vi "VIH - CHM Project - Write TOC File - Add TOC Record - Get Palette Items.vi"(7 "Project Files":T3, 8 "error in":errorcluster, 11 "Palette Menu Path":path) -> (0 "error out":errorcluster, 2 "Items":T2(array[cluster]), 3 "dup Palette Menu Path":path)   [LabVIEW 2014]
doc: "::: VI Helpeks :::\nCopyright (c) 2000-2026 Konstantin Shifershteyn. All rights reserved."
uses:
  _VIH HelpGen - Palette.llb/VIH HelpGen Typedef - Palette - Item Type Enum.ctl
panel:
  # "VI Helpeks\nCopyright (c) 2012-2026 Konstantin Shifershteyn"
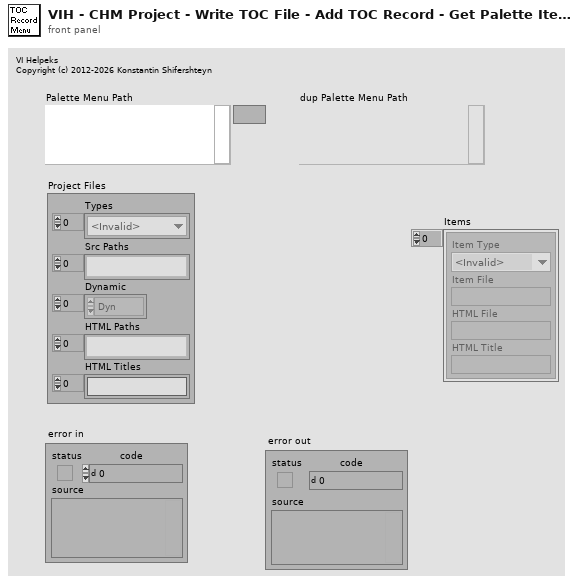
[diagram p1: front panel]
types:
  T1 = typedef "VIH HelpGen Typedef - Palette - Item Type Enum.ctl" = enum32{"<Invalid>", "<unknown>", "VI", "Menu", "LV Func", "Express VI", "Poly VI", "CTL", "HTML"}
  T2 = cluster{"Item Type":T1, "Item File":path, "HTML File":path, "HTML Title":string}[]
  T3 = cluster{"Types":T1[], "Src Paths":path[], "Dynamic":enum16{"Dyn", "Stat", "Both"}[], "HTML Paths":path[], "HTML Titles":string[]}
  T4 = typedef "VIH HelpGen Typedef - Palette - Item Info Cluster.ctl" = cluster{"Item Type":T1, "Item Name":string, "Item File":path, "Parent palette":path, "Not found":bool}
  T5 = cluster{"Item Type":T1, "Item File":path, path, string}
  T6 = cluster{"Item Type":T1, "Item File":path, "HTML File":path, "HTML Title":string}
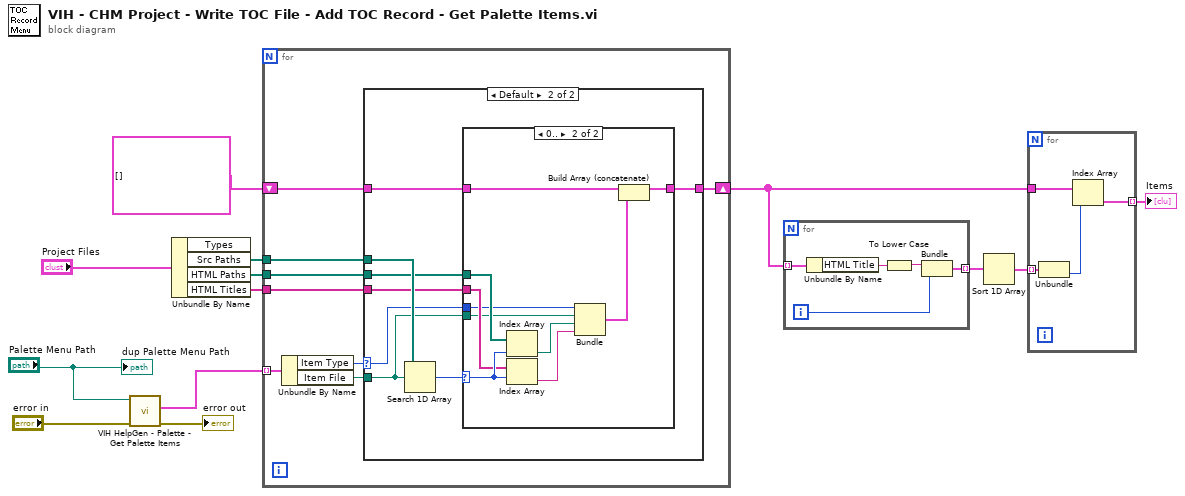
[diagram p0: block diagram]
diagram:
  n1 = call "VIH HelpGen - Palette - Get Palette Items.vi"("error in"="error in", "Palette Path"="Palette Menu Path") -> ("error out"=→"error out":errorcluster, "Items Array"=w10:T4[])  [unwired: 7 in, 1 out]
  n2 = Unbundle By Name("Project Files") -> ("Src Paths"=w9:path[], "HTML Paths"=w6:path[], "HTML Titles"=w7:string[])  [unwired: 1 out]
  n3 = for {
    tunnel: w10 -> [w21] mode=indexing
    tunnel: w9 -> [w18]
    tunnel: w7 -> [w17]
    tunnel: w6 -> [w16]
    shift-right: [w14] -> w3
    shift-left: T2 [] -> [w15]
    n4 = Unbundle By Name(w21) -> ("Item Type"=w20:T1, "Item File"=w19:path)
    n5 = case shown="Default" w20 {
      selector: w20 -> [_ w26]
      tunnel: w19 -> [_ w25]
      tunnel: w18 -> [_ w30]
      tunnel: w17 -> [_ w28]
      tunnel: w16 -> [_ w27]
      tunnel: w15 -> [w22 w24]
      tunnel: [w22 w23] -> w14
      frame "<Invalid>" {
      }
      frame Default {
        n6 = Search 1D Array(1D array=w30, element=w25) -> (index of element=w29:i32)  [unwired: 1 in]
        n7 = case shown="0.." w29 {
          selector: w29 -> [_ w41]
          tunnel: w28 -> [_ w40]
          tunnel: w27 -> [_ w39]
          tunnel: w26 -> [_ w38]
          tunnel: w25 -> [_ w37]
          tunnel: w24 -> [w31 w34]
          tunnel: [w31 w33] -> w23
          frame ..-1 {
          }
          frame 0.. {
            n8 = Index Array(array=w39, index=w41) -> (element=w36:path)
            n9 = Index Array(array=w40, index=w41) -> (element=w35:string)
            n10 = Bundle("Item Type"=w38, "Item File"=w37, w36, w35) -> (w32:T5)  [unwired: 1 in]
            n11 = Build Array (concatenate)(w34, w32) -> (w33:T2)
          }
        }
      }
    }
  }
  n12 = for {
    tunnel: w3 -> [w46] mode=indexing
    tunnel: [w42] -> w4 mode=indexing
    i -> [w43]
    n13 = Unbundle By Name(w46) -> ("HTML Title"=w45:string)
    n14 = To Lower Case(string=w45) -> (all lower case string=w44:string)
    n15 = Bundle(w44, w43) -> (w42:cluster{string, i32})  [unwired: 1 in]
  }
  n16 = Sort 1D Array(array=w4) -> (sorted array=w2:cluster{string, i32}[])
  n17 = for {
    tunnel: w3 -> [w50]
    tunnel: w2 -> [w49] mode=indexing
    tunnel: [w47] -> w1 mode=indexing
    n18 = Unbundle(w49) -> (w48:i32)  [unwired: 1 out]
    n19 = Index Array(array=w50, index=w48) -> (element=w47:T6)
  }
  "Items" <- w1
  "dup Palette Menu Path" <- "Palette Menu Path"
